vi "Var - Context Info.vi"(8 "error in":bool, 11 "VC Handle":T3=-1) -> (0 "error out":bool, 1 "Creator":string, 2 "VC Name":string, 3 "dup VC Handle":T3=-1, 4 "err code":T2 items=["No error", "Invalid variable type", "Variable not found", "Variable already exists", "Invalid context handle", "Input error", "Invalid data format", "No history attached", "History already attached", "Invalid history parameters", "Wrong variable name", "Wrong alias name", "Non-unique alias", "Alias not found", "No alias associated", "Alias already associated", "Wrong context name", "Non-unique context name", "Context name not found", "Invalid parameter", "Generic error", "Memory Full", "Unrecognized LV error", "Unknown error code"], 5 "context life time":T1)   [LabVIEW 2021]
doc: "The VI tests a handle of variables context. If the handle is valid, VI returns a name of the context and a name of the context's creator. See help for this VI for more information.\n\n<B>VC Handle</B> control has to contain a handle to be tested. VI returns an error if the handle doesn't correspond to an opened context.\n\n::: CalcExpress Toolkit :::\nCopyright (c) 2000-2026 Konstantin Shifershteyn. All rights reserved."
uses:
  cetypes.llb/VarMan Variable Context Handle.ctl
  cetypes.llb/VarMan Error Code.ctl
  cetypes.llb/VarMan Context Life Time.ctl
  cersrc/celveng32.dll
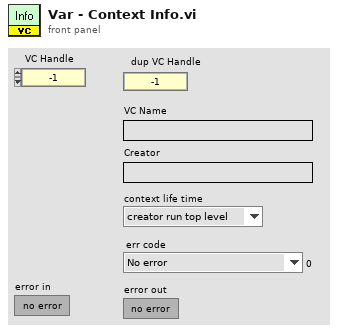
[diagram p1: front panel]
types:
  T1 = typedef "VarMan Context Life Time.ctl" = enum32{"creator run top level", "creator running ", "creator in memory", "untill closed"}
  T2 = typedef "VarMan Error Code.ctl" = u16
  T3 = typedef "VarMan Variable Context Handle.ctl" = i32
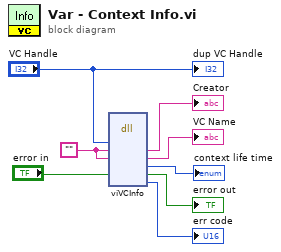
[diagram p0: block diagram]
diagram:
  w8 = ""
  n1 = dll-call lib="C:/LV Projects/CalcExpress 40 LV2021/vi.lib/addons/CalcExpress/cersrc/celveng*.dll" fn="viVCInfo"("vch"="VC Handle", "Creator"=w8, "vcName"=w8, "errf"="error in") -> ("Creator"=→"Creator":string, "vcName"=→"VC Name":string, "context life time"=→"context life time":T1, "errf"=→"error out":bool, "err code"=→"err code":T2)  [unwired: 7 in, 2 out]
  "dup VC Handle" <- "VC Handle"
